vi "Replace Sub VI.vi"(8 "error in (no error)":errorcluster, 11 "VI in":refnum<vi>) -> (0 "error out":errorcluster, 3 "VI out":refnum<vi>)   [LabVIEW 2020, in "Mock Class Generator.lvclass"]
uses:
  Mock Class Generator.lvclass
  <vilib>/Utility/traverseref.llb/TRef TravTarget.ctl
  Mock Class Generator.lvclass/Mock Class Generator.ctl
  <vilib>/Utility/traverseref.llb/VI Scripting - Traverse.lvlib
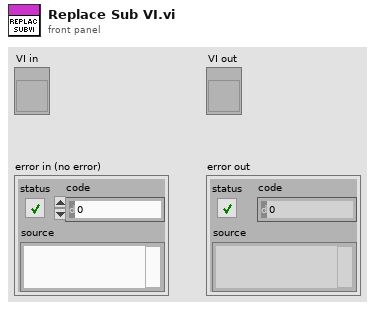
[diagram p1: front panel]
types:
  T1 = typedef "TRef TravTarget.ctl" = enum16{"FP", "BD", "Other"}
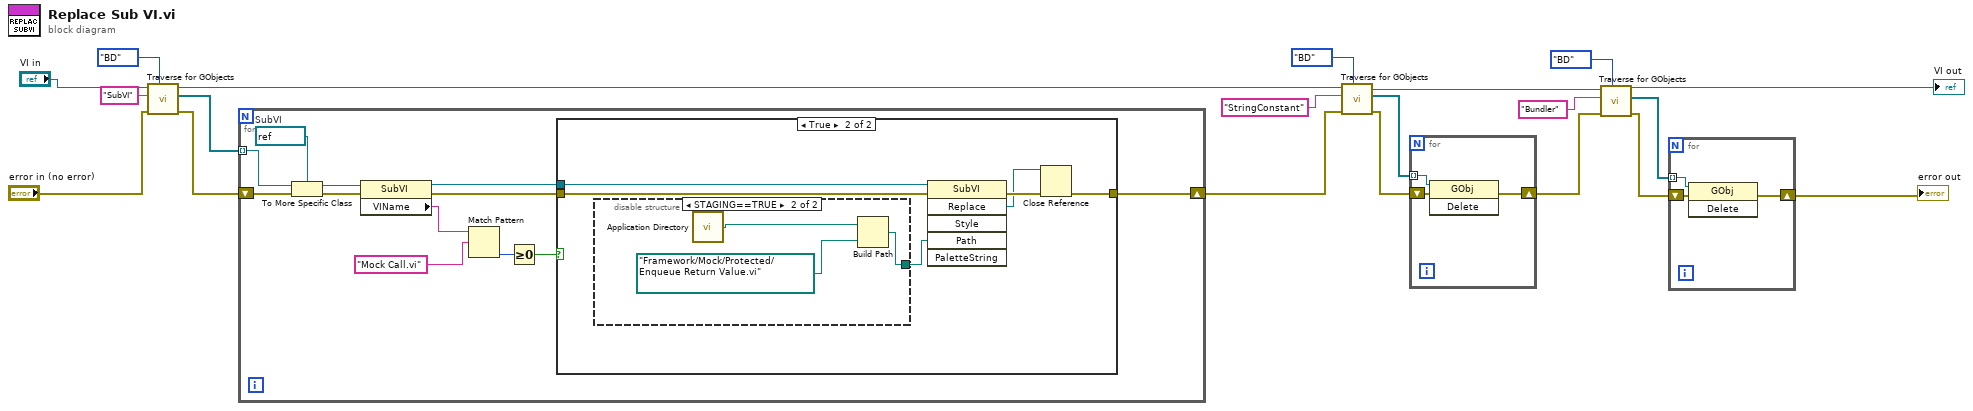
[diagram p0: block diagram]
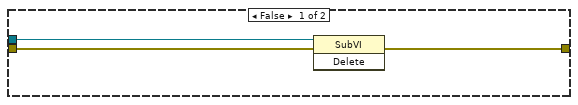
[diagram p2: hidden frame]
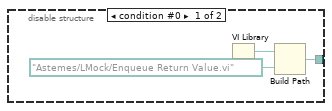
[diagram p3: hidden frame]
diagram:
  n1 = call <vilib>:"Traverse for GObjects.vi"("Traverse Target"=TRef_TravTarget."BD", "error in (no error)"="error in (no error)", "Class Name"="SubVI", "VI Refnum"="VI in") -> ("error out"=w15:errorcluster, "References"=w16:refnum<vi>[], "dup VI Refnum"=w14:refnum<vi>)  [unwired: 4 in, 1 out]
  n2 = for {
    tunnel: w16 -> [w28] mode=indexing
    shift-right: [w21] -> w11
    shift-left: w15 -> [w32]
    w26 = refnum<vi> refnum  # SubVI
    n3 = To More Specific Class(target class=w26, reference=w28, error in=w32) -> (specific class reference=w27:refnum<vi>, error out=w29:errorcluster)
    n4 = property class="SubVI"(reference=w27, error in=w29) -> (reference out=w30:refnum<vi>, error out=w31:errorcluster, "VIName"=w23:string)
    n5 = Match Pattern(string=w23, regular expression="Mock Call.vi") -> (offset past match=w25:i32)  [unwired: 1 in, 3 out]
    n6 = Greater Or Equal To 0?(x=w25) -> (x >= 0?=w24:bool)
    n7 = case shown="True" w24 {
      tunnel: [w33 w37] -> w21
      tunnel: w31 -> [w34 w39]
      tunnel: w30 -> [w35 w38]
      frame False {
        n8 = invoke class="SubVI" method="Delete"(reference=w35, error in=w34) -> (error out=w33:errorcluster)  [unwired: 1 in, 2 out]
      }
      frame True {
        n9 = disable-structure shown="STAGING==TRUE" {
          disable-tunnel: [w42 w45] -> w40
          frame condition #0 {
            n10 = VI Library() -> (path=w43:path)
            n11 = Build Path(base path=w43, name or relative path=path "Astemes/LMock/Enqueue Return Value.vi" ("class path")) -> (appended path=w42:path)
          }
          frame condition #1 (active) {
            n12 = call <vilib>:"Application Directory.vi"() -> ("Application Directory"=w47:path)
            n13 = Build Path(base path=w47, name or relative path=path "Framework/Mock/Protected/Enqueue Return Value.vi" ("appended path")) -> (appended path=w45:path)
          }
        }
        n14 = invoke class="SubVI" method="Replace"(reference=w38, error in=w39, "Path"=w40) -> (error out=w41:errorcluster, "Replace"=w36:refnum<vi>)  [unwired: 3 in, 4 out]
        n15 = Close Reference(reference=w36, error in (no error)=w41) -> (error out=w37:errorcluster)
      }
    }
  }
  n16 = call <vilib>:"Traverse for GObjects.vi"("Traverse Target"=TRef_TravTarget."BD", "error in (no error)"=w11, "Class Name"="StringConstant", "VI Refnum"=w14) -> ("error out"=w10:errorcluster, "References"=w9:refnum<vi>[], "dup VI Refnum"=w4:refnum<vi>)  [unwired: 4 in, 1 out]
  n17 = for {
    shift-right: [w49] -> w3
    shift-left: w10 -> [w50]
    tunnel: w9 -> [w48] mode=indexing
    n18 = invoke class="GObj" method="Delete"(reference=w48, error in=w50) -> (error out=w49:errorcluster)  [unwired: 1 in, 2 out]
  }
  n19 = call <vilib>:"Traverse for GObjects.vi"("Traverse Target"=TRef_TravTarget."BD", "error in (no error)"=w3, "Class Name"="Bundler", "VI Refnum"=w4) -> ("error out"=w7:errorcluster, "References"=w8:refnum<vi>[], "dup VI Refnum"=→"VI out":refnum<vi>)  [unwired: 4 in, 1 out]
  n20 = for {
    shift-right: [w52] -> w2
    shift-left: w7 -> [w53]
    tunnel: w8 -> [w51] mode=indexing
    n21 = invoke class="GObj" method="Delete"(reference=w51, error in=w53) -> (error out=w52:errorcluster)  [unwired: 1 in, 2 out]
  }
  "error out" <- w2
